vi "Handle_Cmd.vi"(8 "error in":errorcluster, 9 "timed out?":bool, 10 "data IN":T1, 11 "FPGA VI Reference IN":refnum<k20>) -> (0 "error out":errorcluster, 3 "FPGA VI Reference IN 2":refnum<k20>)   [LabVIEW 2025]
uses:
  <vilib>/rvi/interface/nirviReadWriteControl/nirviReadWriteControl.xnode
  NiFpgaLv.dll
  <vilib>/Utility/error.llb/Error Cluster From Error Code.vi
  <vilib>/rvi/interface/Simulation/niFpgaSimulationCallBeginRW.vi
  <vilib>/rvi/errors/niLvFpgaAdjustHostInterfaceError.vi
  Command.ctl
  vi/thresholds.ctl
  RT_Cmd.ctl
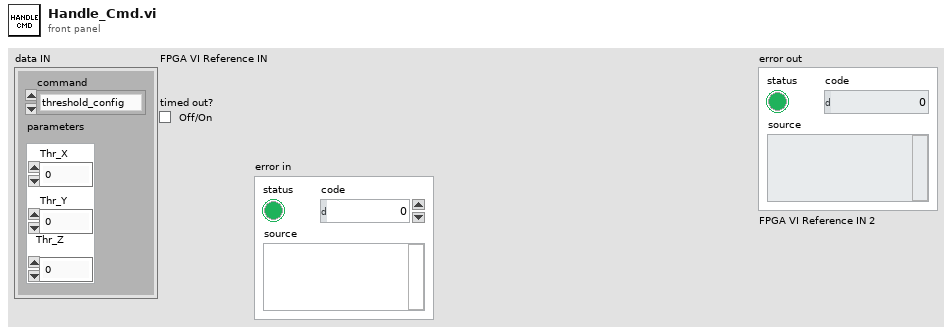
[diagram p1: front panel]
types:
  T1 = typedef "RT_Cmd.ctl" = cluster{"command":T2, "parameters":T3}
  T2 = typedef "Command.ctl" = enum16{"threshold_config", "manual_trigger", "stop"}
  T3 = typedef "thresholds.ctl" = cluster{"Thr_X":i16, "Thr_Y":i16, "Thr_Z":i16}
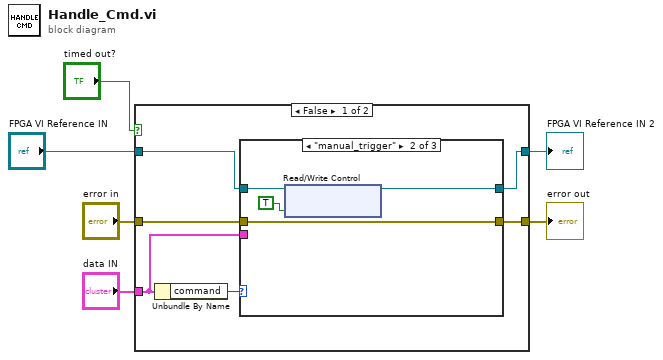
[diagram p0: block diagram]
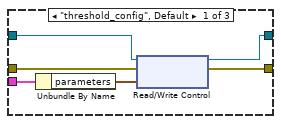
[diagram p2: hidden frame]
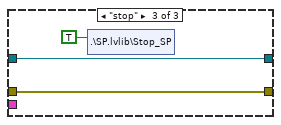
[diagram p3: hidden frame]
diagram:
  n1 = case shown="False" "timed out?" {
    tunnel: "data IN" -> [w11 _]
    tunnel: "FPGA VI Reference IN" -> [w10 w27]
    tunnel: [w9 w27] -> w1
    tunnel: "error in" -> [w8 w26]
    tunnel: [w7 w26] -> w2
    frame False {
      n2 = Unbundle By Name(w11) -> ("command"=w12:T2)
      n3 = case shown="\"manual_trigger\"" w12 {
        tunnel: w11 -> [w18 _ _]
        tunnel: w10 -> [w17 w22 w24]
        tunnel: [w15 w20 w24] -> w9
        tunnel: w8 -> [w14 w19 w23]
        tunnel: [w13 w19 w23] -> w7
        frame "threshold_config", Default {
          n4 = Unbundle By Name(w18) -> ("parameters"=w16:T3)
          n5 = xnode "Read/Write Control"("FPGA VI Reference In"=w17, "error in"=w14, "Threshold"=w16) -> ("FPGA VI Reference Out"=w15:refnum<k20>, "error out"=w13:errorcluster)
        }
        frame "manual_trigger" {
          n6 = xnode "Read/Write Control"("FPGA VI Reference In"=w22, "manual trigger"=TRUE) -> ("FPGA VI Reference Out"=w20:refnum<k20>)  [unwired: 1 in, 1 out]
        }
        frame "stop" {
          n7 = shared-variable ".\\SP.lvlib\\Stop_SP"(TRUE ("Stop_SP")) -> ()  [unwired: 1 in, 1 out]
        }
      }
    }
    frame True {
    }
  }
  "error out" <- w2
  "FPGA VI Reference IN 2" <- w1
